vi "Sample name array for CNAL.vi"(11 "S array":T1(array[cluster])) -> (0 "Sample Sequence array":string[](array[string]), 3 "Sample name array":string[](array[string]))   [LabVIEW 2018]
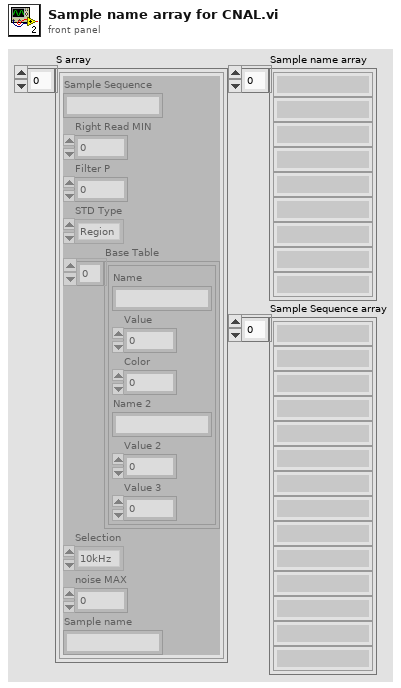
[diagram p1: front panel]
types:
  T1 = cluster{"Sample Sequence":string, "Right Read MIN":i32, "Filter P":i32, "STD Type":enum16{"Region", "Each", "Fixed"}, "Base Table":cluster{"Name":string, "Value":dbl, "Color":u32, "Name 2":string, "Value 2":dbl, "Value 3":dbl}[], "Selection":enum16{"10kHz", "100kHz"}, "noise MAX":i32, "Sample name":string}[]
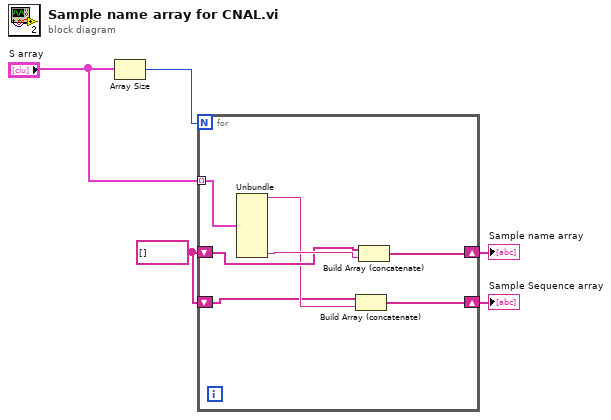
[diagram p0: block diagram]
diagram:
  w1 = string[] []
  n1 = Array Size(array="S array") -> (size(s)=w5:i32)
  n2 = for {
    N: w5 -> [_]
    tunnel: "S array" -> [w12] mode=indexing
    shift-right: [w11] -> w3
    shift-left: w1 -> [w9]
    shift-right: [w7] -> w2
    shift-left: w1 -> [w6]
    n3 = Unbundle(w12) -> ("Sample Sequence"=w8:string, "Sample name"=w10:string)  [unwired: 6 out]
    n4 = Build Array (concatenate)(w6, w8) -> (w7:string[])
    n5 = Build Array (concatenate)(w9, w10) -> (w11:string[])
  }
  "Sample name array" <- w3
  "Sample Sequence array" <- w2
